vi "Test Prepare Path Returns Path Relative to Project Dir.vi"(11 "Test Case In":refnum<class "Report Plugin Test.lvclass">) -> (0 "error out":errorcluster, 3 "Test Case Out":refnum<class "Report Plugin Test.lvclass">)   [LabVIEW 2020, in "Report Plugin Test.lvclass"]
uses:
  Report Plugin Test.lvclass
  Report Plugin Test.lvclass/Report Plugin Test.ctl
  source/Framework/Report Plugin/Report Plugin.lvclass
  bef865c9-9006-4318-9b84-13997f877ae2.vi
  C:/Program Files (x86)/National Instruments/LabVIEW 2020/vi.lib/Astemes/LUnit/Test Case.lvclass
  C:/git/astemes-lunit/source/Framework/Report Plugin/Report Plugin.lvclass
  C:/git/astemes-lunit/source/Framework/Plugin/Plugin.lvclass
  C:/Program Files (x86)/National Instruments/LabVIEW 2020/vi.lib/Astemes/LUnit/LUnit Runnable.lvclass
  C:/git/astemes-lunit/tests/Report Plugin Test/Report Plugin Test.lvclass
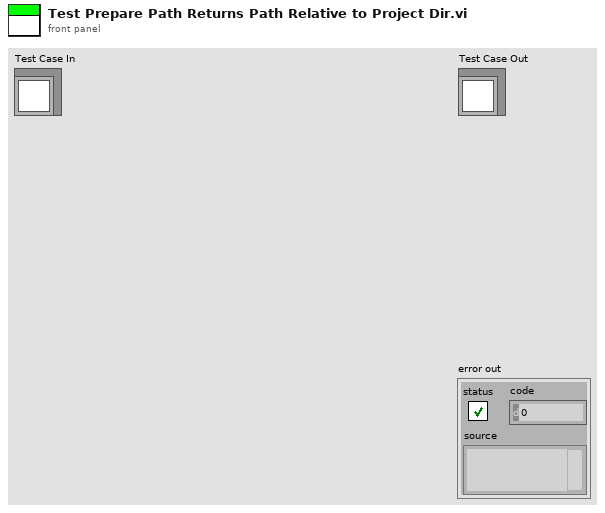
[diagram p1: front panel]
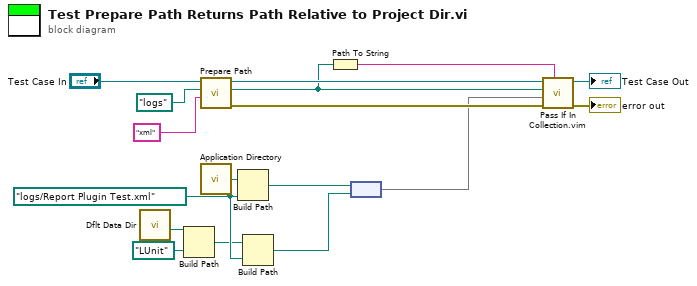
[diagram p0: block diagram]
diagram:
  w6 = path "logs/Report Plugin Test.xml" ("name or relative path")
  n1 = call <vilib>:"Dflt Data Dir.vi"() -> ("App:Default Data Directory"=w2:path)
  n2 = Build Path(base path=w2, name or relative path=path "LUnit") -> (appended path=w3:path)
  n3 = call "Prepare Path.vi"("Extenssion"="xml", "File Path in"=path "logs", "Report Plugin In"="Test Case In") -> ("error out"=w13:errorcluster, "Modified Path"=w5:path, "Report Plugin Out"=w14:refnum<class "Report Plugin Test.lvclass">)  [unwired: 6 in]
  n4 = call <vilib>:"Application Directory.vi"() -> ("Application Directory"=w10:path)
  n5 = Build Path(base path=w10, name or relative path=w6) -> (appended path=w9:path)
  n6 = Build Path(base path=w3, name or relative path=w6) -> (appended path=w8:path)
  n7 = Path To String(path=w5) -> (string=w4:string)
  n8 = node(w9, w8) -> (w7:set{path})
  n9 = call "Pass If In Collection.vim"("Description"=w4, "error in (no error)"=w13, "Collection"=w7, "Expected Element"=w5, "LUnit Test Case In"=w14) -> ("error out"=→"error out":errorcluster, "LUnit Test Case Out"=→"Test Case Out":refnum<class "Report Plugin Test.lvclass">)  [unwired: 5 in]
